vi "SimpleGit-Settings.vi"(11 "path":path) -> ()   [LabVIEW 2017]
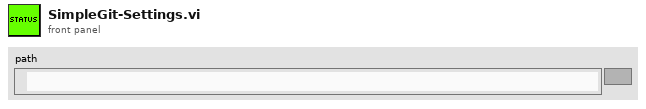
[diagram p1: front panel]
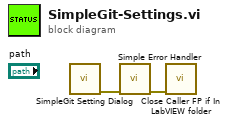
[diagram p0: block diagram]
diagram:
  n1 = call "SimpleGit Setting Dialog.vi"() -> ("error out"=w1:errorcluster)  [unwired: 11 in]
  n2 = call <vilib>:"Simple Error Handler.vi"("error in (no error)"=w1) -> ("error out"=w2:errorcluster)  [unwired: 4 in, 4 out]
  n3 = call "Close Caller FP if In LabVIEW folder.vi"("error in (no error)"=w2) -> ()  [unwired: 10 in, 1 out]
